vi "layout.vi"(0 "reference":refnum<class "ChoiceNode.lvclass">, 1 "graph":refnum<class "Graph.lvclass">, 2 "graphics":refnum<class "Graphics.lvclass">, 3 "grid":refnum<class "Grid.lvclass">, 5 "error in (no error)":errorcluster) -> (14 "reference out":refnum<class "ChoiceNode.lvclass">, 19 "error out":errorcluster)   [LabVIEW 2020, in "ChoiceNode.lvclass"]
doc: "public void layout(Graph g, Graphics2D g2, Grid grid)"
uses:
  <resource>/Framework/Providers/Open_GDS/UML/ChoiceNode_class/ChoiceNode.lvclass
  C:/Program Files (x86)/National Instruments/LabVIEW 2020/resource/Framework/Providers/Open_GDS/UML/RectangularNode_class/RectangularNode.lvclass
  <resource>/Framework/Providers/Open_GDS/UML/Graph_class/Graph.lvclass
  <resource>/Framework/Providers/Open_GDS/UML/Graphics_class/Graphics.lvclass
  <resource>/Framework/Providers/Open_GDS/UML/Grid_class/Grid.lvclass
  <resource>/Framework/Providers/Open_GDS/UML/General/Rectangle/Rectangle Rectangle2D.ctl
  <resource>/Framework/Providers/Open_GDS/UML/MultiLineString_class/MultiLineString.lvclass
  <resource>/Framework/Providers/Open_GDS/UML/RectangularNode_class/RectangularNode.lvclass
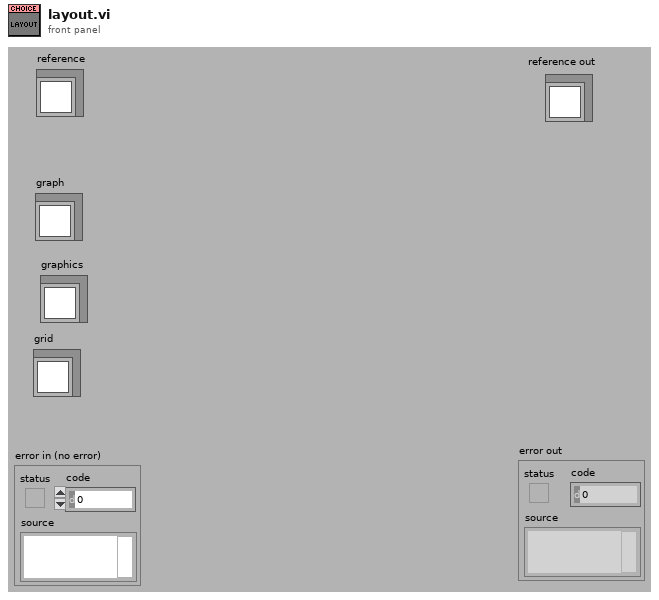
[diagram p1: front panel]
types:
  T1 = typedef "Rectangle Rectangle2D.ctl" = cluster{"x":dbl, "y":dbl, "width":dbl, "height":dbl}
  T2 = typedef "ChoiceNode.lvclass/ObjectAttributes.ctl" = cluster{"Text":refnum<class "MultiLineString.lvclass">, "DEFAULT_WIDTH":i32, "DEFAULT_HEIGHT":i32}
  T3 = typedef "RectangularNode.lvclass/ObjectAttributes.ctl" = cluster{"bounds":T1}
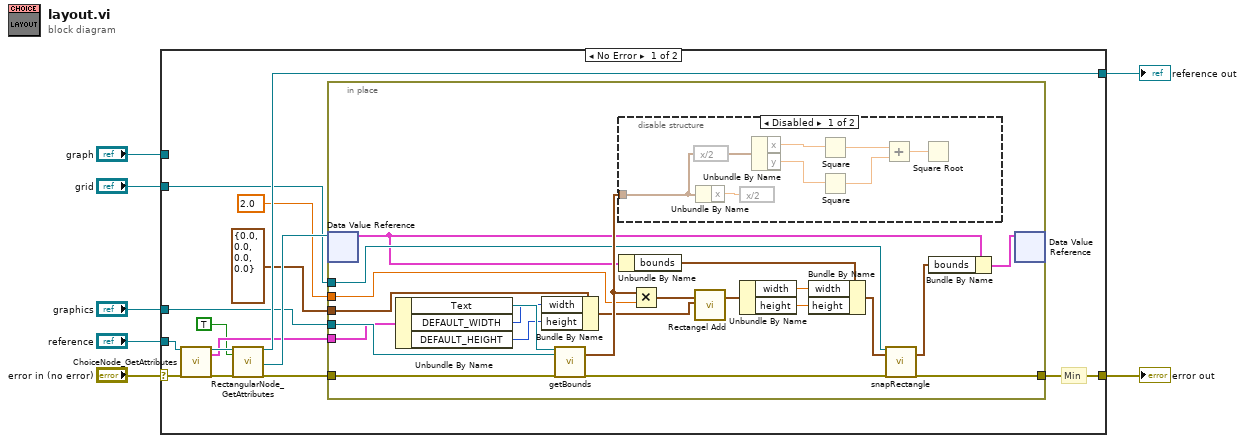
[diagram p0: block diagram]
diagram:
  n1 = case shown="No Error" "error in (no error)" {
    selector: "error in (no error)" -> [w19 w52]
    tunnel: "reference" -> [w21 w53]
    tunnel: [w10 w52] -> w6
    tunnel: [w20 w53] -> w5
    tunnel: "graph" -> [_ _]
    tunnel: "graphics" -> [w15 _]
    tunnel: "grid" -> [w11 _]
    frame No Error {
      # "Min"
      n2 = call <resource>:"ChoiceNode_GetAttributes.vi"("reference in"=w21, "error in (no error)"=w19) -> ("reference out"=w18:refnum<class "ChoiceNode.lvclass">, "Data"=w9:T2, "error out"=w17:errorcluster)  [unwired: 14 in, 1 out]
      n3 = call <resource>:"RectangularNode_GetAttributes.vi"("reference in"=w18, "OnlyGetDvrReference(False)"=TRUE, "error in (no error)"=w17) -> ("reference out"=w20:refnum<class "ChoiceNode.lvclass">, "DataRef"=w16:refnum<data-value>, "error out"=w14:errorcluster)  [unwired: 13 in, 1 out]
      n4 = in-place {
        in-place-border: w15 -> [w40]
        in-place-border: w14 -> [w39]
        in-place-border: T1 {"x"=0.0, "y"=0.0, "width"=0.0, "height"=0.0} ("bounds") -> [w36]
        in-place-border: 2.0 ("x") -> [w34]
        in-place-border: w11 -> [w32]
        in-place-border: [w29] -> w10
        in-place-border: w9 -> [w22]
        n5 = in-place-dvr #1(w16) -> (w24:T3)  [unwired: 1 out]
        n6 = Unbundle By Name(w22) -> ("Text"=w43:refnum<class "MultiLineString.lvclass">, "DEFAULT_WIDTH"=w42:i32, "DEFAULT_HEIGHT"=w41:i32)
        n7 = Bundle By Name(cluster=w36, "width"=w42, "height"=w41) -> (w35:T1)
        n8 = call-dynamic "getBounds.vi"("reference"=w43, "graphics"=w40, "error in (no error)"=w39) -> ("bounds"=w38:T1, "error out"=w37:errorcluster)  [unwired: 15 out]
        n9 = disable-structure shown="Disabled" {
          disable-tunnel: w38 -> [w50 _]
          frame Disabled {
            n10 = expression code="x/2"(w50) -> (w49:T1)
            n11 = Unbundle By Name(w50) -> ("x"=w51:dbl)
            n12 = expression code="x/2"(w51) -> ()  [unwired: 1 out]
            n13 = Unbundle By Name(w49) -> ("x"=w48:dbl, "y"=w47:dbl)
            n14 = Square(x=w48) -> (x^2=w46:dbl)
            n15 = Square(x=w47) -> (x^2=w45:dbl)
            n16 = Add(x=w46, y=w45) -> (x+y=w44:dbl)
            n17 = Square Root(x=w44) -> ()  [unwired: 1 out]
          }
          frame Enabled {
          }
        }
        n18 = Unbundle By Name(w24) -> ("bounds"=w27:T1)
        n19 = Multiply(x=w38, y=w34) -> (x*y=w33:T1)
        n20 = call <resource>:"Rectangel Add.vi"("bounds1"=w33, "bounds2"=w35) -> ("boundsAdded"=w28:T1)  [unwired: 3 in, 14 out]
        n21 = Unbundle By Name(w28) -> ("width"=w26:dbl, "height"=w25:dbl)
        n22 = Bundle By Name(cluster=w27, "width"=w26, "height"=w25) -> (w31:T1)
        n23 = call <resource>:"snapRectangle.vi"("reference"=w32, "bounds"=w31, "error in (no error)"=w37) -> ("boundsOut"=w30:T1, "error out"=w29:errorcluster)  [unwired: 15 out]
        n24 = Bundle By Name(cluster=w24, "bounds"=w30) -> (w23:T3)
        n25 = in-place-dvr #1(w23) -> ()  [unwired: 2 out]
      }
    }
    frame Error {
    }
  }
  "reference out" <- w5
  "error out" <- w6
